vi "draw.vi"(0 "reference":refnum<class "StateNode.lvclass">, 1 "graphics":refnum<class "Graphics.lvclass">, 5 "error in (no error)":errorcluster) -> (14 "reference out":refnum<class "StateNode.lvclass">, 19 "error out":errorcluster)   [LabVIEW 2020, in "StateNode.lvclass"]
doc: "public void draw(Graphics2D g2, Point2D p, Point2D q)"
uses:
  <resource>/Framework/Providers/Open_GDS/UML/StateNode_class/StateNode.lvclass
  C:/Program Files (x86)/National Instruments/LabVIEW 2020/resource/Framework/Providers/Open_GDS/UML/RectangularNode_class/RectangularNode.lvclass
  <resource>/Framework/Providers/Open_GDS/UML/Graphics_class/Graphics.lvclass
  <resource>/Framework/Providers/Open_GDS/UML/General/Point/Point Point2D.ctl
  <resource>/Framework/Providers/Open_GDS/UML/UMLEditor/UMLEditor_StoredColors.ctl
  <resource>/Framework/Providers/Open_GDS/UML/MultiLineString_class/MultiLineString.lvclass
  <resource>/Framework/Providers/Open_GDS/UML/RectangularNode_class/RectangularNode.lvclass
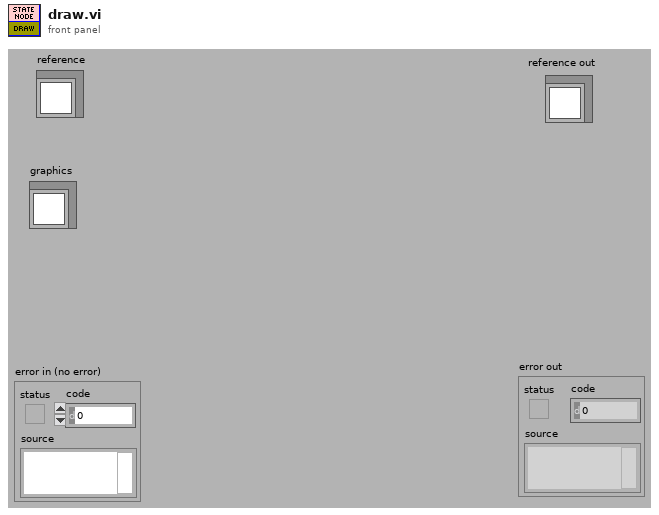
[diagram p1: front panel]
types:
  T1 = typedef "UMLEditor_StoredColors.ctl" = enum16{"ClassBackgroudColor", "ClassBackgroudColorWithClassPath", "ClassBackgroudColorForApplicationVIStereotype", "ClassBackgroudColorForTypeStereotype", "StateBackgroudColor", "ClassBackgroudColorForInterfaceStereotype"}
  T2 = typedef "Point Point2D.ctl" = cluster{"x":dbl, "y":dbl}
  T3 = typedef "StateNode.lvclass/ObjectAttributes.ctl" = cluster{"state":refnum<class "MultiLineString.lvclass">, "action":refnum<class "MultiLineString.lvclass">, "DEFAULT_WIDTH":i32, "DEFAULT_HEIGHT":i32}
  T4 = typedef "RectangularNode.lvclass/ObjectAttributes.ctl" = cluster{"bounds":T5}
  T5 = typedef "Rectangle Rectangle2D.ctl" = cluster{"x":dbl, "y":dbl, "width":dbl, "height":dbl}
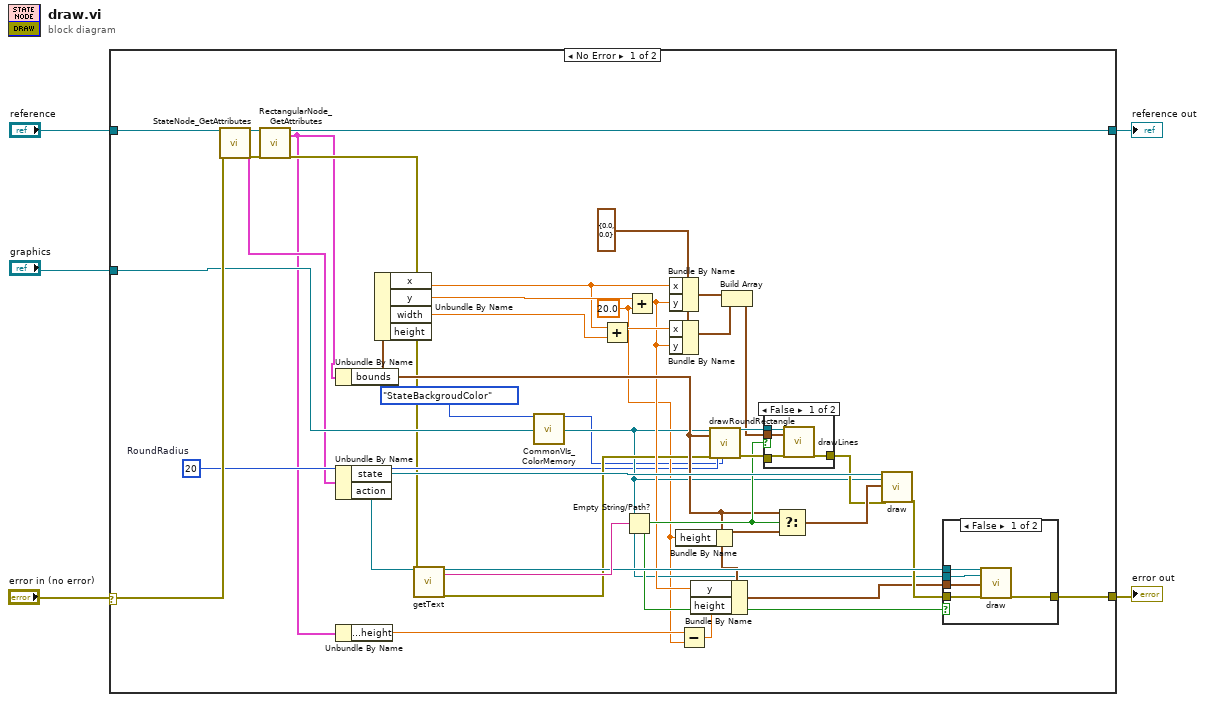
[diagram p0: block diagram]
diagram:
  n1 = case shown="No Error" "error in (no error)" {
    selector: "error in (no error)" -> [w21 w56]
    tunnel: "reference" -> [w44 w57]
    tunnel: [w20 w56] -> w4
    tunnel: [w7 w57] -> w3
    tunnel: "graphics" -> [w18 _]
    frame No Error {
      w14 = i16 20  # RoundRadius
      w32 = T2 {"x"=0.0, "y"=0.0} ("point2D")
      w15 = 20.0 ("y")
      n2 = call <resource>:"StateNode_GetAttributes.vi"("reference in"=w44, "error in (no error)"=w21) -> ("reference out"=w10:refnum<class "StateNode.lvclass">, "Data"=w11:T3, "error out"=w9:errorcluster)  [unwired: 1 in, 14 out]
      n3 = call <resource>:"RectangularNode_GetAttributes.vi"("reference in"=w10, "error in (no error)"=w9) -> ("reference out"=w7:refnum<class "StateNode.lvclass">, "Data"=w6:T4, "error out"=w8:errorcluster)  [unwired: 14 in, 1 out]
      n4 = Unbundle By Name(w6) -> ("bounds"=w24:T5)
      n5 = Unbundle By Name(w11) -> ("state"=w43:refnum<class "MultiLineString.lvclass">, "action"=w42:refnum<class "MultiLineString.lvclass">)
      n6 = Unbundle By Name(w6) -> ("bounds.height"=w17:dbl)
      n7 = Unbundle By Name(w24) -> ("x"=w31:dbl, "y"=w33:dbl, "width"=w30:dbl)  [unwired: 1 out]
      n8 = call-dynamic "getText.vi"("reference"=w42, "error in (no error)"=w8) -> ("reference out"=w39:refnum<class "MultiLineString.lvclass">, "text"=w41:string, "error out"=w22:errorcluster)  [unwired: 15 in]
      n9 = call <resource>:"CommonVIs_ColorMemory.vi"("ColorName"=UMLEditor_StoredColors."StateBackgroudColor" ("UMLPathes")) -> ("Color Out"=w12:u32)  [unwired: 3 in, 15 out]
      n10 = Add(x=w31, y=w30) -> (x+y=w29:dbl)
      n11 = Empty String/Path?(string/path=w41) -> (empty?=w35:bool)
      n12 = Add(x=w33, y=w15) -> (x+y=w23:dbl)
      n13 = Bundle By Name(cluster=w32, "x"=w31, "y"=w23) -> (w28:T2)
      n14 = Bundle By Name(cluster=w32, "x"=w29, "y"=w23) -> (w27:T2)
      n15 = Bundle By Name(cluster=w24, "height"=w15) -> (w25:T5)
      n16 = Subtract(x=w17, y=w15) -> (x-y=w16:dbl)
      n17 = Bundle By Name(cluster=w24, "y"=w23, "height"=w16) -> (w19:T5)
      n18 = call-dynamic "drawRoundRectangle.vi"("reference"=w18, "rectangle"=w24, "error in (no error)"=w22, "RoundRadius"=w14, "FillClor(if not used=BorderColorIsUsed,AutoFill)"=w12) -> ("reference out"=w37:refnum<class "Graphics.lvclass">, "error out"=w36:errorcluster)  [unwired: 13 in]
      n19 = Build Array(w28, w27) -> (w26:T2[])
      n20 = case shown="False" w35 {
        tunnel: w37 -> [w48 _]
        tunnel: w36 -> [w47 w49]
        tunnel: [w46 w49] -> w34
        tunnel: w26 -> [w45 _]
        frame False {
          n21 = call <resource>:"drawLines.vi"("reference"=w48, "points"=w45, "error in (no error)"=w47) -> ("error out"=w46:errorcluster)  [unwired: 4 in, 12 out]
        }
        frame True {
        }
      }
      n22 = Select(t=w24, s=w35, f=w25) -> (s? t:f=w40:T5)
      n23 = call-dynamic "draw.vi"("reference"=w43, "graphics"=w18, "bounds"=w40, "error in (no error)"=w34) -> ("error out"=w38:errorcluster)  [unwired: 14 in, 1 out]
      n24 = case shown="False" w35 {
        tunnel: w39 -> [w54 _]
        tunnel: w18 -> [w53 _]
        tunnel: w38 -> [w52 w55]
        tunnel: [w51 w55] -> w20
        tunnel: w19 -> [w50 _]
        frame False {
          n25 = call-dynamic "draw.vi"("reference"=w54, "graphics"=w53, "bounds"=w50, "error in (no error)"=w52) -> ("error out"=w51:errorcluster)  [unwired: 14 in, 1 out]
        }
        frame True {
        }
      }
    }
    frame Error {
    }
  }
  "reference out" <- w3
  "error out" <- w4
